vi "MQTT Properties - Encode.vi"(7 "MQTT Properties":T1[](array[typedef]) {"Property" items=["Payload Format Indicator"=1, "Message Expiry Interval"=2, "Content Type"=3, "Response Topic"=8, "Correlation Data"=9, "Subscription Identifier"=11, "Session Expiry Interval"=17, "Assigned Client Identifier"=18, "Server Keep Alive"=19, "Authentication Method"=21, "Authentication Data"=22, "Request Problem Information"=23, "Will Delay Interval"=24, "Request Response Information"=25, "Response Information"=26, "Server Reference"=28, "Reason String"=31, "Receive Maximum"=33, "Topic Alias Maximum"=34, "Topic Alias"=35, "Maximum QoS"=36, "Retain Available"=37, "User Property"=38, "Maximum Packet Size"=39, "Wildcard Subscription Available"=40, "Subscription Identifier Available"=41, "Shared Subscription Available"=42]}, 11 "error in (no error)":errorcluster) -> (8 "Encoded MQTT Properties":u8[](array[numeric]), 15 "error out":errorcluster)   [LabVIEW 2019, in "KoRE-MQTT.lvlib"]
doc: "Copyright (c) 2025 KoRElibs.com\nSPDX-License-Identifier: EUPL-1.2\n\nThis VI is licensed under the European Union Public License (EUPL) Version 1.2. You may use this VI unmodified in proprietary works. If you distribute a modified version of this file, the modified file must be released under the EUPL-1.2. Full license: https://joinup.ec.europa.eu/asset/eupl/eupl/1.2/"
uses:
  KoRE-MQTT.lvlib
  Public/TypeDefs/MQTT Property - GENERIC.ctl
  Public/TypeDefs/MQTT Property Type.ctl
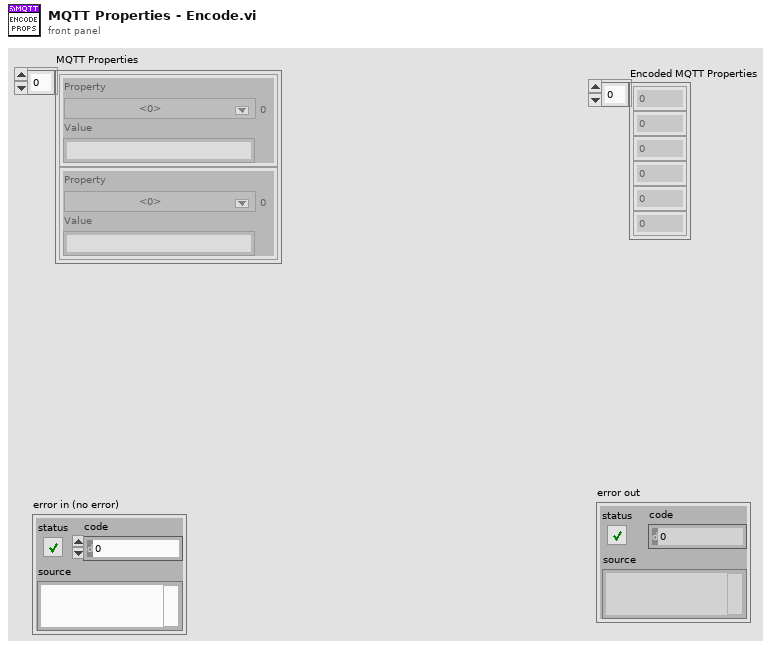
[diagram p1: front panel]
types:
  T1 = typedef "KoRE-MQTT.lvlib/MQTT Property - GENERIC.ctl" = cluster{"Property":T2, "Value":string}
  T2 = typedef "KoRE-MQTT.lvlib/MQTT Property Type.ctl" = u8
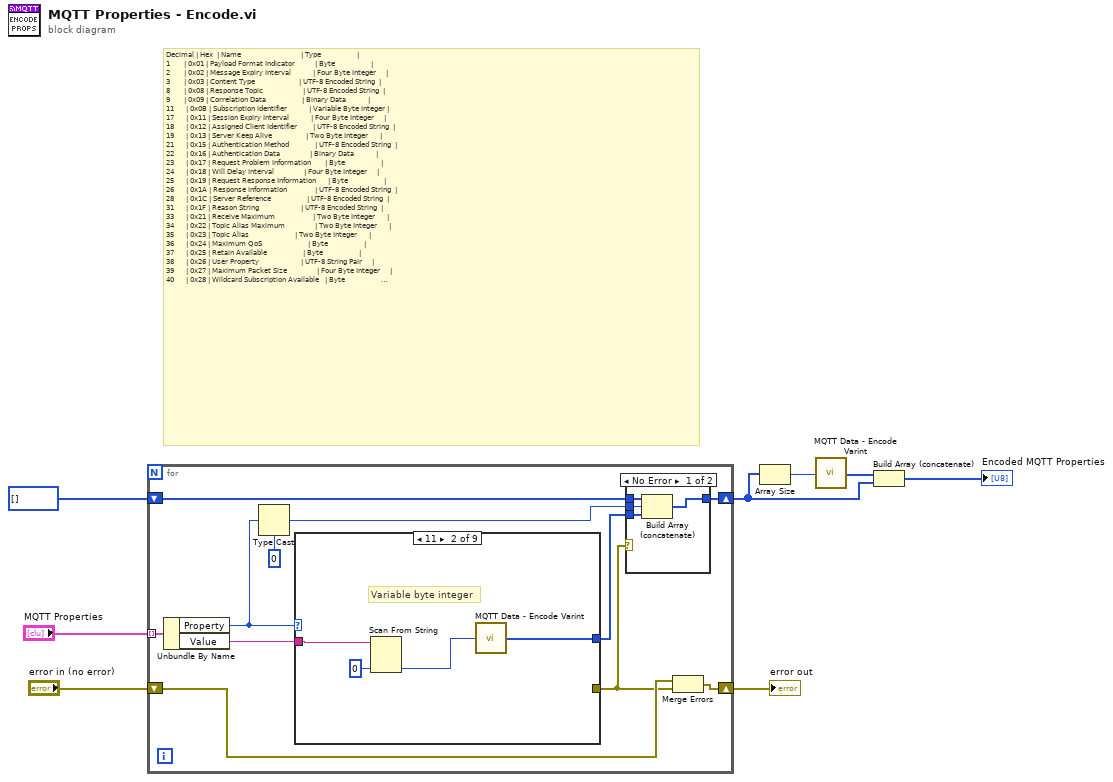
[diagram p0: block diagram]
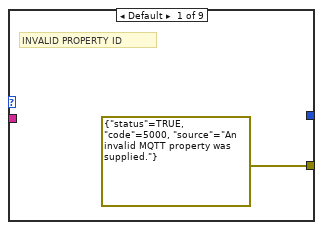
[diagram p3: hidden frame]
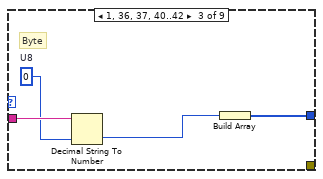
[diagram p4: hidden frame]
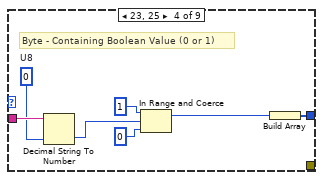
[diagram p5: hidden frame]
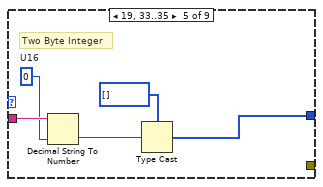
[diagram p6: hidden frame]
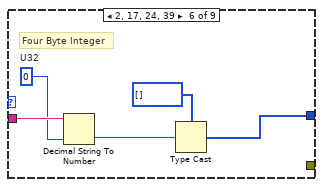
[diagram p7: hidden frame]
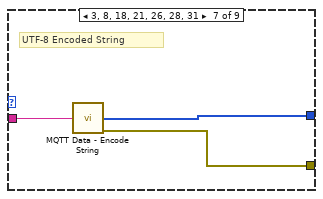
[diagram p8: hidden frame]
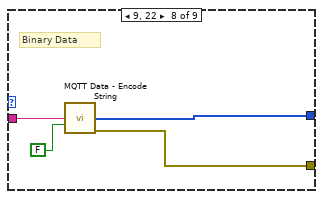
[diagram p9: hidden frame]
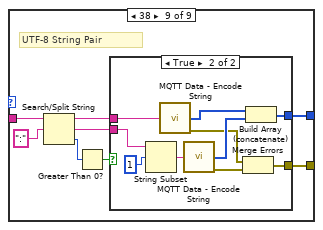
[diagram p10: hidden frame]
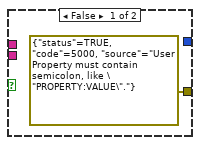
[diagram p11: hidden frame]
diagram:
  # "Decimal | Hex  | Name                              | Type                  |\n1       | 0x01 | Payload Format Indicator          | Byte                  |\n2       | 0x02 | Message Expiry Interval           | Four Byte Integer     |\n3       | 0x03 | Content Type                      | UTF-8 Encoded String  |\n8       | 0x08 | Response Topic                    | UTF-8 Encoded String  |\n9       | 0x09 | Correlation Data                  | Binary Data           |\n11      | 0x0B | Subscription Identifier           | Variable Byte Integer |\n17      | 0x11 | Session Expiry Interval           | Four Byte Integer     |\n18      | 0x12 | Assigned Client Identifier        | UTF-8 Encoded String  |\n19      | 0x13 | Server Keep Alive                 | Two Byte Integer      |\n21      | 0x15 | Authentication Method             | UTF-8 Encoded String  |\n22      | 0x16 | Authentication Data               | Binary Data           |\n23      | 0x17 | Request Problem Information       | Byte                  |\n24      | 0x18 | Will Delay Interval               | Four Byte Integer     |\n25      | 0x19 | Request Response Information      | Byte                  |\n26      | 0x1A | Response Information              | UTF-8 Encoded String  |\n28      | 0x1C | Server Reference                  | UTF-8 Encoded String  |\n31      | 0x1F | Reason String                     | UTF-8 Encoded String  |\n33      | 0x21 | Receive Maximum                   | Two Byte Integer      |\n34      | 0x22 | Topic Alias Maximum               | Two Byte Integer      |\n35      | 0x23 | Topic Alias                       | Two Byte Integer      |\n36      | 0x24 | Maximum QoS                       | Byte                  |\n37      | 0x25 | Retain Available                  | Byte                  |\n38      | 0x26 | User Property                     | UTF-8 String Pair     |\n39      | 0x27 | Maximum Packet Size               | Four Byte Integer     |\n40      | 0x28 | Wildcard Subscription Available   | Byte                  |\n41      | 0x29 | Subscription Identifier Available | Byte                  |\n42      | 0x2A | Shared Subscription Available     | Byte                  |"
  n1 = for {
    tunnel: "MQTT Properties" -> [w19] mode=indexing
    shift-right: [w17] -> w5
    shift-left: u8[] [] ("appended array") -> [w16]
    shift-right: [w11] -> w1
    shift-left: "error in (no error)" -> [w10]
    n2 = Unbundle By Name(w19) -> ("Property"=w15:T2, "Value"=w18:string)
    n3 = Type Cast(type=u8 0, x=w15) -> (*(type *) &x=w13:u8)
    n4 = case shown="11" w15 {
      tunnel: w18 -> [_ w28 w33 w40 w44 w49 w53 w57 w65]
      tunnel: [_ w29 w30 w39 w43 w48 w52 w56 w59] -> w12
      tunnel: [errorcluster {"status"=TRUE, "code"=5000, "source"="An invalid MQTT property was supplied."} ("error out") _ _ _ _ _ w51 w55 w58] -> w9
      frame Default {
        # "INVALID PROPERTY ID"
      }
      frame 11 {
        # "Variable byte integer"
        n5 = Scan From String(input string=w28, default 1=u32 0 ("default value 14")) -> (output 1=w26:u32)  [unwired: 3 in, 3 out]
        n6 = call "MQTT Data - Encode Varint.vi"("Value"=w26) -> ("encoded value"=w29:u8[])  [unwired: 14 in]
      }
      frame 1, 36, 37, 40..42 {
        w32 = u8 0  # U8
        # "Byte"
        n7 = Decimal String To Number(string=w33, default (0L)=w32) -> (number=w31:u8)  [unwired: 1 in, 1 out]
        n8 = Build Array(w31) -> (w30:u8[])
      }
      frame 23, 25 {
        w35 = u8 0  # U8
        # "Byte - Containing Boolean Value (0 or 1)"
        n9 = Decimal String To Number(string=w40, default (0L)=w35) -> (number=w38:u8)  [unwired: 1 in, 1 out]
        n10 = In Range and Coerce(upper limit=u8 1, x=w38, lower limit=u8 0) -> (coerced(x)=w34:u8)  [unwired: 1 out]
        n11 = Build Array(w34) -> (w39:u8[])
      }
      frame 19, 33..35 {
        w42 = u16 0  # U16
        # "Two Byte Integer"
        n12 = Decimal String To Number(string=w44, default (0L)=w42) -> (number=w41:u16)  [unwired: 1 in, 1 out]
        n13 = Type Cast(type=u8[] [], x=w41) -> (*(type *) &x=w43:u8[])
      }
      frame 2, 17, 24, 39 {
        w47 = u32 0  # U32
        # "Four Byte Integer"
        n14 = Decimal String To Number(string=w49, default (0L)=w47) -> (number=w46:u32)  [unwired: 1 in, 1 out]
        n15 = Type Cast(type=u8[] [], x=w46) -> (*(type *) &x=w48:u8[])
      }
      frame 3, 8, 18, 21, 26, 28, 31 {
        # "UTF-8 Encoded String"
        n16 = call "MQTT Data - Encode String.vi"("String in"=w53) -> ("Bytes out"=w52:u8[], "error out"=w51:errorcluster)  [unwired: 13 in]
      }
      frame 9, 22 {
        # "Binary Data"
        n17 = call "MQTT Data - Encode String.vi"("String in"=w57, "To UTF-8?"=FALSE ("UTF-8")) -> ("Bytes out"=w56:u8[], "error out"=w55:errorcluster)  [unwired: 12 in]
      }
      frame 38 {
        # "UTF-8 String Pair"
        n18 = Search/Split String(string=w65, search string/char (-)=":") -> (substring before match=w61:string, match + rest of string=w60:string, offset of match=w63:i32)  [unwired: 1 in]
        n19 = Greater Than 0?(x=w63) -> (x > 0?=w62:bool)
        n20 = case shown="True" w62 {
          tunnel: w61 -> [_ w76]
          tunnel: w60 -> [_ w69]
          tunnel: [_ w73] -> w59
          tunnel: [errorcluster {"status"=TRUE, "code"=5000, "source"="User Property must contain semicolon, like \"PROPERTY:VALUE\"."} ("error out") w72] -> w58
          frame False {
          }
          frame True {
            n21 = String Subset(string=w69, offset (0)=1) -> (substring=w68:string)  [unwired: 1 in]
            n22 = call "MQTT Data - Encode String.vi"("String in"=w76) -> ("Bytes out"=w75:u8[], "error out"=w71:errorcluster)  [unwired: 13 in]
            n23 = call "MQTT Data - Encode String.vi"("String in"=w68) -> ("Bytes out"=w74:u8[], "error out"=w70:errorcluster)  [unwired: 13 in]
            n24 = Merge Errors(w71, w70) -> (w72:errorcluster)
            n25 = Build Array (concatenate)(w75, w74) -> (w73:u8[])
          }
        }
      }
    }
    n26 = case shown="No Error" w9 {
      tunnel: [w23 w24] -> w17
      tunnel: w16 -> [w22 w24]
      tunnel: w13 -> [w21 _]
      tunnel: w12 -> [w20 _]
      frame No Error {
        n27 = Build Array (concatenate)(w22, w21, w20) -> (w23:u8[])
      }
      frame Error {
      }
    }
    n28 = Merge Errors(w10, w9) -> (w11:errorcluster)
  }
  "error out" <- w1
  n29 = Array Size(array=w5) -> (size(s)=w7:i32)
  n30 = call "MQTT Data - Encode Varint.vi"("Value"=w7) -> ("encoded value"=w6:u8[])  [unwired: 14 in]
  n31 = Build Array (concatenate)(w6, w5) -> (→"Encoded MQTT Properties":u8[])
